vi "Test Runner Error Codes.vi"(8 "error in (no error)":errorcluster) -> (0 "error out":errorcluster)   [LabVIEW 2020]
uses:
  classes/Test Runner.Folder/Test Runner.Folder.lvclass
  C:/projects/caraya/src/classes/Test Runner/Test Runner.lvclass
  classes/Test Runner/Test Runner.lvclass/Test Runner.ctl
  classes/Assert/Assert Equal Value_Variant.vi
  classes/Test/Test.lvclass
  classes/Assert/Assert.lvclass
  classes/Test Runner/Test Runner.lvclass
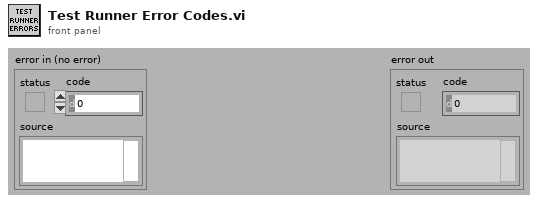
[diagram p1: front panel]
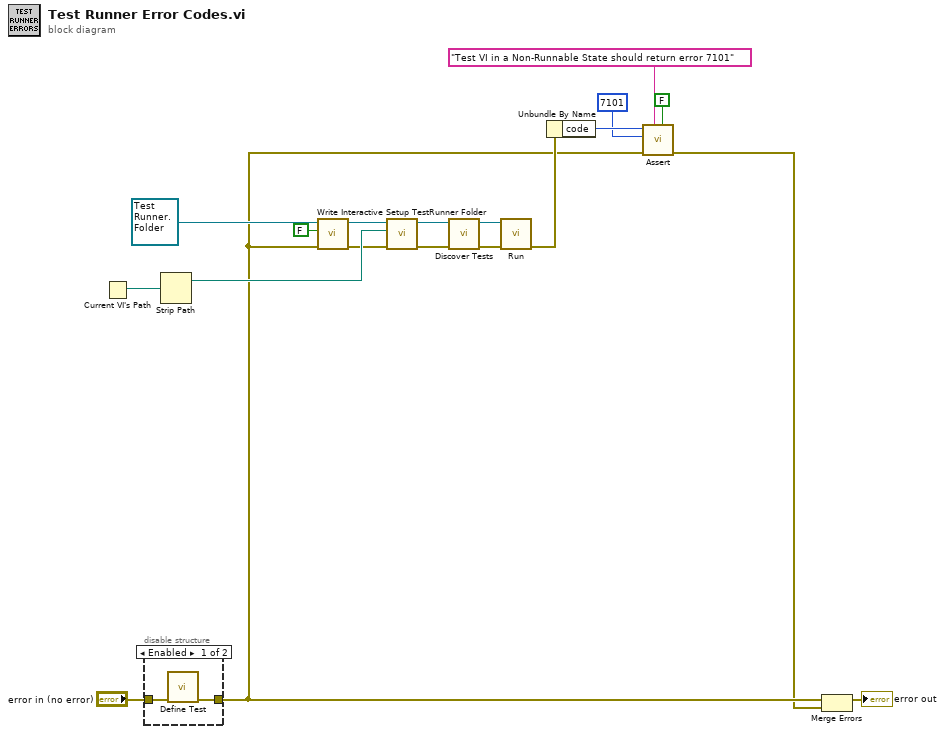
[diagram p0: block diagram]
diagram:
  n1 = Current VI's Path() -> (path=w14:path)
  n2 = disable-structure shown="Enabled" {
    disable-tunnel: "error in (no error)" -> [w20 w21]
    disable-tunnel: [w19 w21] -> w4
    frame Enabled {
      n3 = call "Define Test.vi"("error in (no error)"=w20) -> ("error out"=w19:errorcluster)  [unwired: 9 in, 1 out]
    }
    frame Disabled {
    }
  }
  n4 = Strip Path(path=w14) -> (stripped path=w13:path)  [unwired: 1 out]
  n5 = call "Write Interactive.vi"("Interactive"=FALSE, "Test Runner in"=refnum<class "Test Runner.Folder.lvclass"> refnum ("Caraya.lvlib:Test Runner.Folder.lvclass")) -> ("Test Runner out"=w12:refnum<class "Test Runner.Folder.lvclass">)  [unwired: 9 in]
  n6 = call "Setup TestRunner Folder.vi"("error in (no error)"=w4, "Directory to search"=w13, "Test Runner.Folder"=w12) -> ("error out"=w15:errorcluster, "Test Runner.Folder out"=w16:refnum<class "Test Runner.Folder.lvclass">)  [unwired: 7 in]
  n7 = call "Discover Tests.vi"("error in (no error)"=w15, "Test Runner in"=w16) -> ("error out"=w9:errorcluster, "Test Runner out"=w8:refnum<class "Test Runner.Folder.lvclass">)  [unwired: 8 in]
  n8 = call "Run.vi"("error in (no error)"=w9, "Test Runner in"=w8) -> ("error out"=w7:errorcluster)  [unwired: 7 in, 2 out]
  n9 = Unbundle By Name(w7) -> ("code"=w6:i32)
  n10 = call-poly "Assert.vi"("Assert Only? (F)"=FALSE, "Label"="Test VI in a Non-Runnable State should return error 7101", "error in (no error)"=w4, "Y"=7101 ("code"), "X"=w6) -> ("error out"=w3:errorcluster)  [unwired: 5 in, 1 out]
  n11 = Merge Errors(w4, w3) -> (→"error out":errorcluster)
